vi "GMAP_API_Configure (SubVI).vi"(8 "error in":errorcluster, 11 "Browser control in":refnum<vi>) -> (0 "error out":errorcluster, 2 "Event Registration Refnum":refnum<event-registration>, 3 "Browser control out":refnum<vi>)   [LabVIEW 2025]
doc: "This VI initializes and configures WebView browser\non a LabVIEW front panel"
uses:
  <vilib>/sklein/WebView2 XControl/WebView2 XControl/WebView2 Control.xctl
  <vilib>/sklein/WebView2/Webview2 Lib/WebView2 Control Object/Events.ctl
  <vilib>/sklein/WebView2/Webview2 Lib/WebView2 Control Object/Navigation Event Data.ctl
  <vilib>/sklein/WebView2/Webview2 Lib/WebView2 Control Object/Source Changed Event Data.ctl
  <vilib>/sklein/WebView2/Webview2 Lib/WebView2 Control Object/Navigation Start Event Data.ctl
  <vilib>/sklein/WebView2/Webview2 Lib/WebView2 Control Object/Paths.ctl
  <vilib>/sklein/WebView2/Webview2 Lib/WebView2 Control Object/WebView2 Control.lvclass
panel:
  out "Paths":T1
  # "This VI initializes and configures WebView browser\non a LabVIEW front panel"
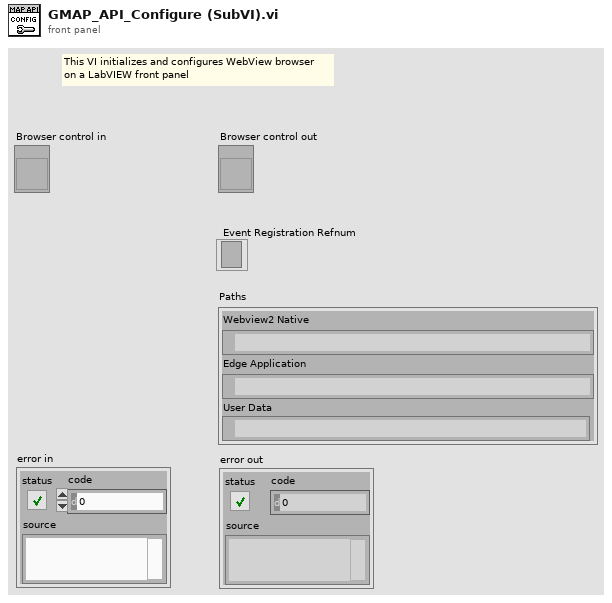
[diagram p1: front panel]
types:
  T1 = typedef "WebView2.lvlib/WebView2 Control.lvclass/Paths.ctl" = cluster{"Webview2 Native":path, "Edge Application":path, "User Data":path}
  T2 = typedef "WebView2.lvlib/WebView2 Control.lvclass/Events.ctl" = cluster{"Navigation Complete Event":refnum<user-event>, "Source Changed Event":refnum<user-event>, "Document Title Changed Event":refnum<user-event>, "Status Bar Text Changed":refnum<user-event>, "Web Message Received":refnum<user-event>, "Window Close Requested":refnum<user-event>, "DOM Loaded":refnum<user-event>, "Navigation Started Event":refnum<user-event>}
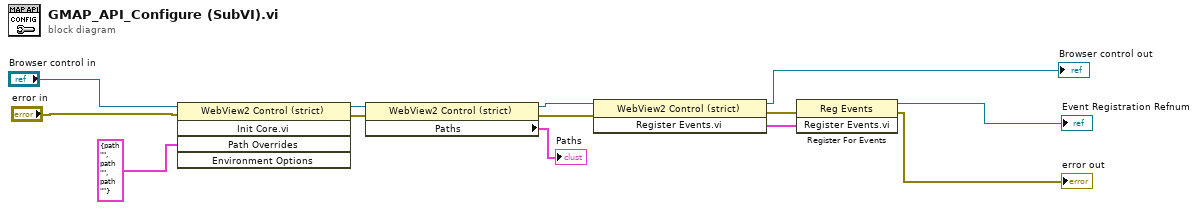
[diagram p0: block diagram]
diagram:
  n1 = invoke class="WebView2 Control (strict)" method="Init Core.vi"(reference="Browser control in", error in="error in", "Path Overrides"=T1 {"Webview2 Native"=path "", "Edge Application"=path "", "User Data"=path ""}) -> (reference out=w7:refnum<vi>, error out=w6:errorcluster)  [unwired: 2 in, 3 out]
  n2 = property class="WebView2 Control (strict)"(reference=w7, error in=w6) -> (reference out=w2:refnum<vi>, error out=w1:errorcluster, "Paths"=→"Paths":T1)
  n3 = invoke class="WebView2 Control (strict)" method="Register Events.vi"(reference=w2, error in=w1) -> (reference out=→"Browser control out":refnum<vi>, error out=w11:errorcluster, "Register Events.vi"=w12:T2)  [unwired: 1 in]
  n4 = register-events(error in=w11, w12) -> (reference out=→"Event Registration Refnum":refnum<event-registration>, error out=→"error out":errorcluster)  [unwired: 1 in]
